vi "Read subModule.vi"(8 "error in":errorcluster, 10 "XML Path":path) -> (0 "error out":errorcluster, 1 "PLC":T2={"PLC Folder Names"=[["Station0_Rx", "OP50A_TesterRxSignals"], ["Station0_Tx", "OP50A_TesterTxSignals"], ["Station1_Rx", "OP50B_TesterRxSignals"], ["Station1_Tx", "OP50B_TesterTxSignals"], ["Station2_Rx", "OP60A_TesterRxSignals"], ["Station2_Tx", "OP60A_TesterTxSignals"], ["Station3_Rx", "OP60B_TesterRxSignals"], ["Station3_Tx", "OP60B_TesterTxSignals"], ["Station4_Rx", "OP70A_TesterRxSignals"], ["Station4_Tx", "OP70A_TesterTxSignals"], ["Station5_Rx", "OP70B_TesterRxSignals"], ["Station5_Tx", "OP70B_TesterTxSignals"]], "PLC URL"="opc.tcp://localhost:49580 ", "Ignition Folder Names"=[["Ignition0_Rx", "[Submodule_EOL]/StaA/TesterRx"], ["Ignition0_Tx", "[Submodule_EOL]/StaA/TesterTx"], ["Ignition1_Rx", "[Submodule_EOL]/StaB/TesterRx"], ["Ignition1_Tx", "[Submodule_EOL]/StaB/TesterTx"], ["Ignition2_Rx", "[Submodule_EOL]/StaC/TesterRx"], ["Ignition2_Tx", "[Submodule_EOL]/StaC/TesterTx"], ["Ignition3_Rx", "[Submodule_EOL]/StaD/TesterRx"], ["Ignition3_Tx", "[Submodule_EOL]/StaD/TesterTx"], ["Ignition4_Rx", "[Submodule_EOL]/StaE/TesterRx"], ["Ignition4_Tx", "[Submodule_EOL]/StaE/TesterTx"], ["Ignition5_Rx", "[Submodule_EOL]/StaF/TesterRx"], ["Ignition5_Tx", "[Submodule_EOL]/StaF/TesterTx"]], "Ignition URL"="opc.tcp://10.64.0.22:62541/discovery", "Test Name"="Battery Submodule EOL"}, 2 "Instrument":T1, 3 "Setting":T3={"Local Database"="JungDB", "Connect OPC Trial"=0, "Timeout Connect OPC"=0.0, "AbstractUUT Path"="C:\\Working copy\\Battery-Submodule-EOL-OOP\\Sequence\\OPC UA Client\\OPC UA\\Abstract.lvclass", "PreUUT Path"="C:\\Working copy\\Battery-Submodule-EOL-OOP\\Sequence\\OPC UA Client\\OPC UA\\Abstract.lvclass", "Test Path"="C:\\Working copy\\Battery-Submodule-EOL-OOP\\Sequence\\OPC UA Client\\TestExec\\TestExec.lvclass", "PostUUT Path"="C:\\Working copy\\Battery-Submodule-EOL-OOP\\Sequence\\OPC UA Client\\PostUUT\\PostUUT.lvclass"} {"Timeout Connect OPC" format="%#_f"})   [LabVIEW 2025, in "Submodule EOL.lvlib" / "Submodule EOL configuration.lvclass"]
uses:
  Submodule EOL configuration/Submodule EOL configuration.lvclass
  Submodule EOL configuration/Setting.ctl
  Submodule EOL configuration/PLC.ctl
  Submodule EOL configuration/Instrumnet.ctl
  Users/Public/Documents/Sandia National Labs/TSS Plugin/CEF.lvlibp
  Users/Public/Documents/Sandia National Labs/TSS Plugin/CEF.lvlibp/serializable configuration/CEF_serializable configuration.lvclass
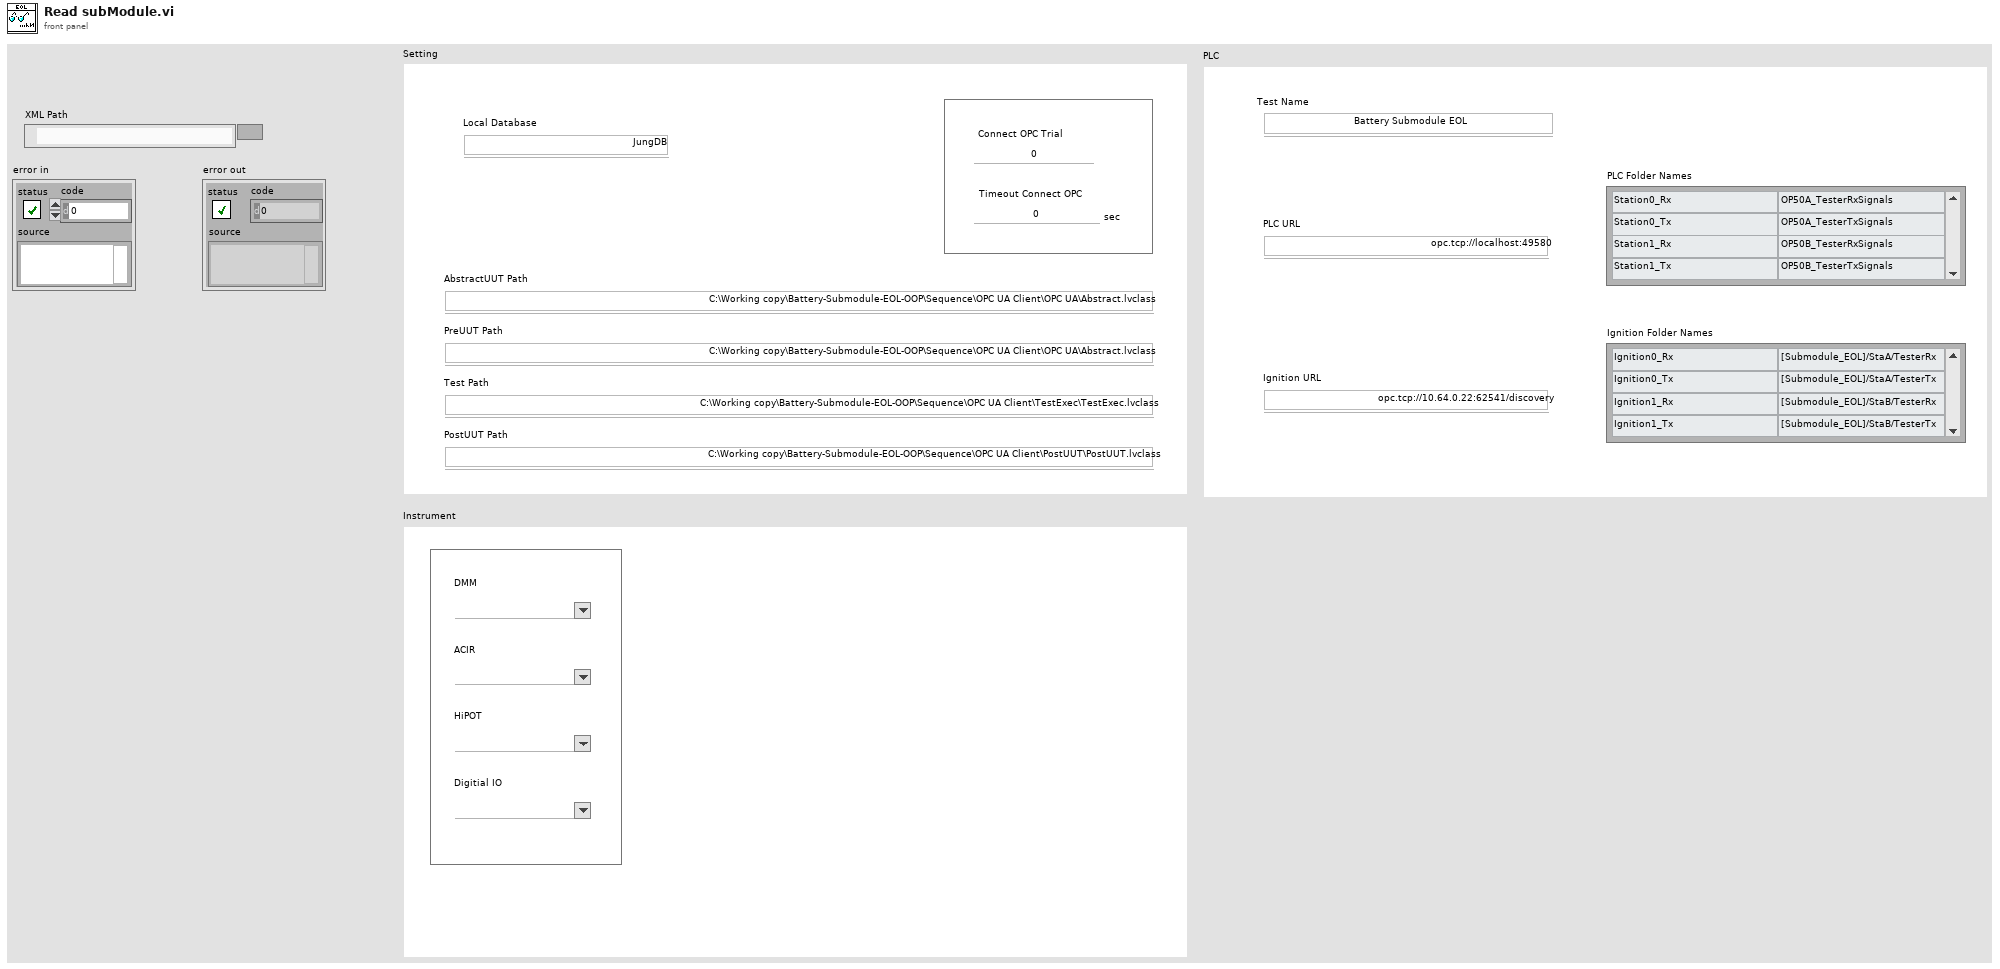
[diagram p1: front panel]
types:
  T1 = typedef "Submodule EOL.lvlib/Submodule EOL configuration.lvclass/Instrumnet.ctl" = cluster{"Digitial IO":string, "HiPOT":string, "ACIR":string, "DMM":string}
  T2 = typedef "Submodule EOL.lvlib/Submodule EOL configuration.lvclass/PLC.ctl" = cluster{"PLC Folder Names":string[][], "PLC URL":string, "Ignition Folder Names":string[][], "Ignition URL":string, "Test Name":string}
  T3 = typedef "Submodule EOL.lvlib/Submodule EOL configuration.lvclass/Setting.ctl" = cluster{"Local Database":string, "Connect OPC Trial":u32, "Timeout Connect OPC":dbl, "AbstractUUT Path":string, "PreUUT Path":string, "Test Path":string, "PostUUT Path":string}
  T4 = cluster{"hierarchy structure":cluster{"root":string, "hierarchy":cluster{"current node":string, "children":string[]}[]}, "instance data":cluster{"ID":string, "Alias":string, "class":string, "version":string, "data":string}[]}
  T5 = cluster{"ID":string, "Alias":string, "class":string, "version":string, "data":string}[]
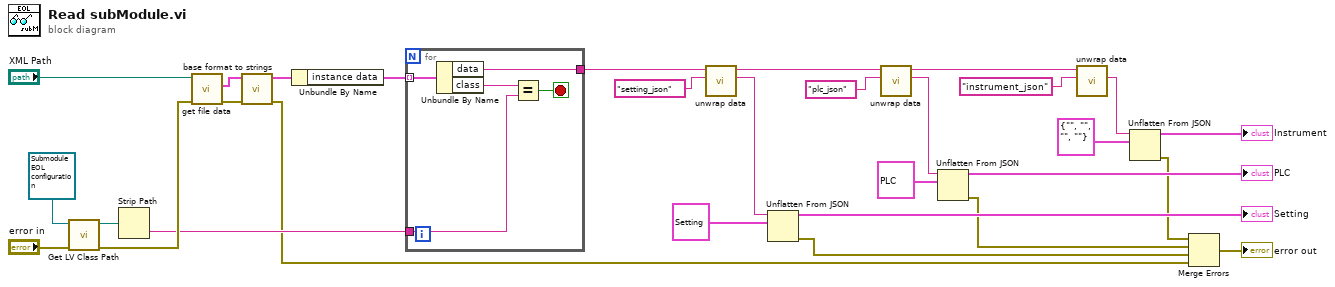
[diagram p0: block diagram]
diagram:
  n1 = call <vilib>:"Get LV Class Path.vi"("error in (no error)"="error in", "object"=refnum<class "Submodule EOL configuration.lvclass"> refnum ("Submodule EOL.lvlib:Submodule config")) -> ("error out"=w5:errorcluster, "class path"=w6:path)  [unwired: 8 in]
  n2 = Strip Path(path=w6) -> (name=w4:string)  [unwired: 1 out]
  n3 = call "get file data.vi"("error in"=w5, "Path"="XML Path") -> ("error out"=w24:errorcluster, "format"=w25:cluster{"version":string, "data":string})  [unwired: 8 in]
  n4 = call "base format to strings.vi"("error in"=w24, "format"=w25) -> ("error out"=w3:errorcluster, "data"=w23:T4)  [unwired: 8 in]
  n5 = Unbundle By Name(w23) -> ("instance data"=w8:T5)
  n6 = for {
    tunnel: w8 -> [w35] mode=indexing
    tunnel: w4 -> [w31]
    tunnel: [w33] -> w7
    stop <- w34 stop-if-true
    n7 = Unbundle By Name(w35) -> ("data"=w33:string, "class"=w32:string)
    n8 = Equal?(x=w32, y=w31) -> (x = y?=w34:bool)
  }
  n9 = call "unwrap data.vi"("identifier"="setting_json" ("additional identifier"), "data to unwrap"=w7) -> ("unwrapped data"=w13:string, "remaining string"=w15:string)  [unwired: 8 in]
  n10 = Unflatten From JSON(JSON string=w13, type and defaults=T3 {"Local Database"="opc.tcp://localhost:49580 ", "Connect OPC Trial"=3, "Timeout Connect OPC"=5.0, "AbstractUUT Path"="opc.tcp://localhost:49580 ", "PreUUT Path"="opc.tcp://10.64.0.22:62541/discovery", "Test Path"="opc.tcp://10.64.0.22:62541/discovery", "PostUUT Path"="Battery Submodule EOL"} ("Event")) -> (value=→"Setting":T3, error out=w11:errorcluster)  [unwired: 5 in]
  n11 = call "unwrap data.vi"("identifier"="plc_json" ("additional identifier"), "data to unwrap"=w15) -> ("unwrapped data"=w17:string, "remaining string"=w19:string)  [unwired: 8 in]
  n12 = Unflatten From JSON(JSON string=w17, type and defaults=T2 {"PLC Folder Names"=[["Station0_Rx", "OP50A_TesterRxSignals"], ["Station0_Tx", "OP50A_TesterTxSignals"], ["Station1_Rx", "OP50B_TesterRxSignals"], ["Station1_Tx", "OP50B_TesterTxSignals"], ["Station2_Rx", "OP60A_TesterRxSignals"], ["Station2_Tx", "OP60A_TesterTxSignals"], ["Station3_Rx", "OP60B_TesterRxSignals"], ["Station3_Tx", "OP60B_TesterTxSignals"], ["Station4_Rx", "OP70A_TesterRxSignals"], ["Station4_Tx", "OP70A_TesterTxSignals"], ["Station5_Rx", "OP70B_TesterRxSignals"], ["Station5_Tx", "OP70B_TesterTxSignals"]], "PLC URL"="opc.tcp://localhost:49580 ", "Ignition Folder Names"=[["Ignition0_Rx", "[Submodule_EOL]/StaA/TesterRx"], ["Ignition0_Tx", "[Submodule_EOL]/StaA/TesterTx"], ["Ignition1_Rx", "[Submodule_EOL]/StaB/TesterRx"], ["Ignition1_Tx", "[Submodule_EOL]/StaB/TesterTx"], ["Ignition2_Rx", "[Submodule_EOL]/StaC/TesterRx"], ["Ignition2_Tx", "[Submodule_EOL]/StaC/TesterTx"], ["Ignition3_Rx", "[Submodule_EOL]/StaD/TesterRx"], ["Ignition3_Tx", "[Submodule_EOL]/StaD/TesterTx"], ["Ignition4_Rx", "[Submodule_EOL]/StaE/TesterRx"], ["Ignition4_Tx", "[Submodule_EOL]/StaE/TesterTx"], ["Ignition5_Rx", "[Submodule_EOL]/StaF/TesterRx"], ["Ignition5_Tx", "[Submodule_EOL]/StaF/TesterTx"]], "Ignition URL"="opc.tcp://10.64.0.22:62541/discovery", "Test Name"="Battery Submodule EOL"} ("PLC")) -> (value=→"PLC":T2, error out=w10:errorcluster)  [unwired: 5 in]
  n13 = call "unwrap data.vi"("identifier"="instrument_json" ("additional identifier"), "data to unwrap"=w19) -> ("unwrapped data"=w21:string)  [unwired: 8 in, 1 out]
  n14 = Unflatten From JSON(JSON string=w21, type and defaults=T1 {"Digitial IO"="", "HiPOT"="", "ACIR"="", "DMM"=""} ("Instrument")) -> (value=→"Instrument":T1, error out=w9:errorcluster)  [unwired: 5 in]
  n15 = Merge Errors(w9, w10, w11, w3) -> (→"error out":errorcluster)
